vi "路灯仿真_B站参考版V1.vi"() -> ()   [LabVIEW 2014]
panel:
  in  "布尔":bool
  out "计时器":dbl
  out "绿":bool
  out "黄":bool
  out "红":bool
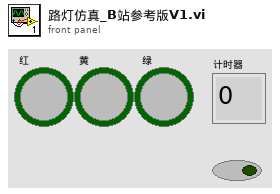
[diagram p1: front panel]
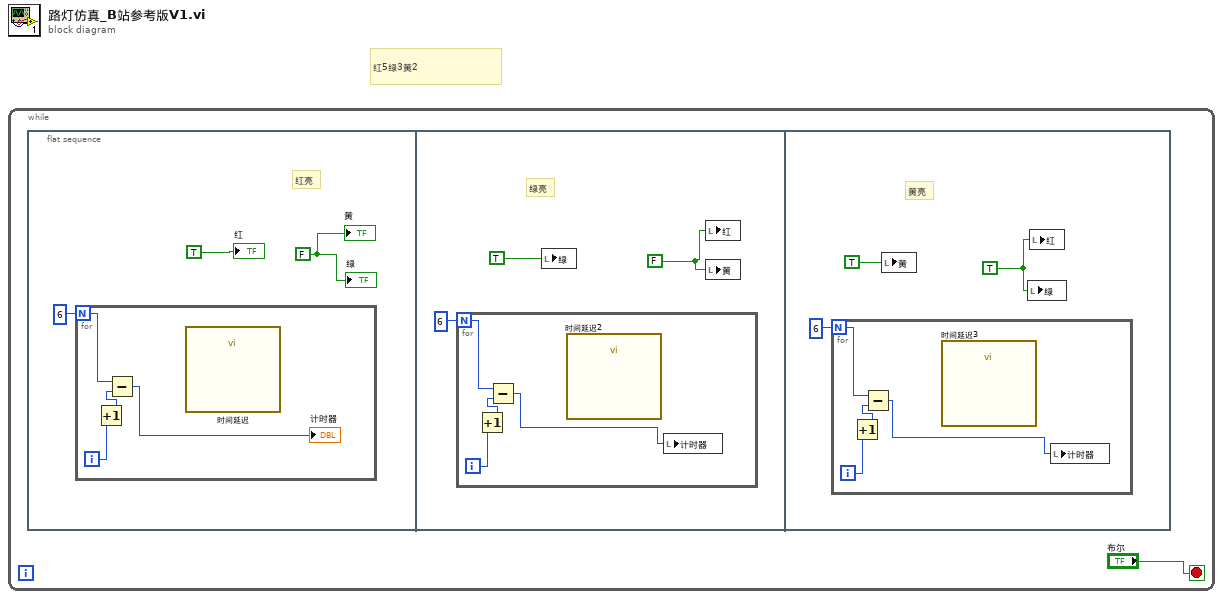
[diagram p0: block diagram]
diagram:
  # "红5绿3黄2"
  n1 = while {
    stop <- "布尔" stop-if-true
    n2 = flat-sequence {
      frame #0 {
        w3 = FALSE
        # "红亮"
        n3 = for {
          N: 6 -> [w8]
          i -> [w5]
          n4 = Increment(x=w5) -> (x+1=w6:i32)
          n5 = Subtract(x=w8, y=w6) -> (x-y=→"计时器":i32)
          n6 = call "时间延迟"() -> ()  [unwired: 11 in, 1 out]
        }
        "红" <- TRUE
        "黄" <- w3
        "绿" <- w3
      }
      frame #1 {
        w11 = FALSE
        # "绿亮"
        n7 = for {
          N: 6 -> [w15]
          i -> [w13]
          n8 = Increment(x=w13) -> (x+1=w14:i32)
          n9 = Subtract(x=w15, y=w14) -> (x-y=w12:i32)
          n10 = call "时间延迟2"() -> ()  [unwired: 11 in, 1 out]
          n11 = local write "计时器"(w12) -> ()
        }
        n12 = local write "绿"(TRUE) -> ()
        n13 = local write "红"(w11) -> ()
        n14 = local write "黄"(w11) -> ()
      }
      frame #2 {
        w18 = TRUE
        # "黄亮"
        n15 = for {
          N: 6 -> [w22]
          i -> [w20]
          n16 = Increment(x=w20) -> (x+1=w21:i32)
          n17 = Subtract(x=w22, y=w21) -> (x-y=w19:i32)
          n18 = call "时间延迟3"() -> ()  [unwired: 11 in, 1 out]
          n19 = local write "计时器"(w19) -> ()
        }
        n20 = local write "黄"(TRUE) -> ()
        n21 = local write "绿"(w18) -> ()
        n22 = local write "红"(w18) -> ()
      }
    }
  }
